vi "Get XNET Signal Names.vi"(6 "Add Info?":bool, 7 "Parent Ref in":T1 format="%.0x", 8 "error in":errorcluster, 9 "Tree In":refnum<vi>, 10 "Parent":string, 11 "Frms":refnum<k21>[](array[refnum])) -> (0 "error out":errorcluster, 1 "Tree Out":refnum<vi>, 3 "XNET Signal Names":refnum<k21>[](array[refnum]))   [LabVIEW 2015, in "Protection and Counter Addon System Explorer.lvlib"]
uses:
  Protection and Counter Addon System Explorer.lvlib
  <vilib>/NI Veristand/Custom Device API/Custom Device Item Ref.ctl
  <vilib>/NI Veristand/Custom Device API/Custom Device Channel.ctl
  <vilib>/NI Veristand/Custom Device API/Custom Device Channel Type.ctl
  Shared/SubVIs/GUID Lookup.vi
  <vilib>/NI Veristand/Custom Device API/Set Item Property (U32).vi
  <resource>/objmgr/xnet.rc
  <vilib>/NI VeriStand/Custom Device API/Custom Device API.lvlib
  Shared/Protection and Counter Addon Shared.lvlib
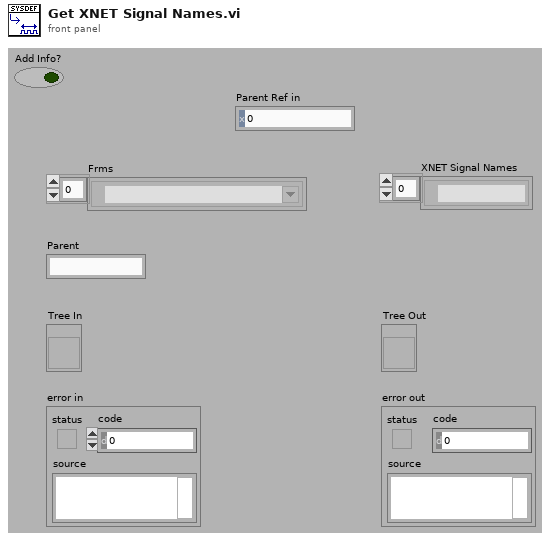
[diagram p1: front panel]
types:
  T1 = typedef "Custom Device API.lvlib/Custom Device Item Ref.ctl" = u64
  T2 = typedef "Custom Device API.lvlib/Custom Device Channel.ctl" = cluster{"Type":T3, "Units":string, "Default Value":dbl, "Faultable":bool, "Scalable":bool}
  T3 = typedef "Custom Device API.lvlib/Custom Device Channel Type.ctl" = enum16{"Input", "Output"}
  T4 = typedef "Custom Device API.lvlib/Custom Device Item Info.ctl" = cluster{"Name":string, "Is Channel":bool, "GUID":string, "Is Waveform":bool}
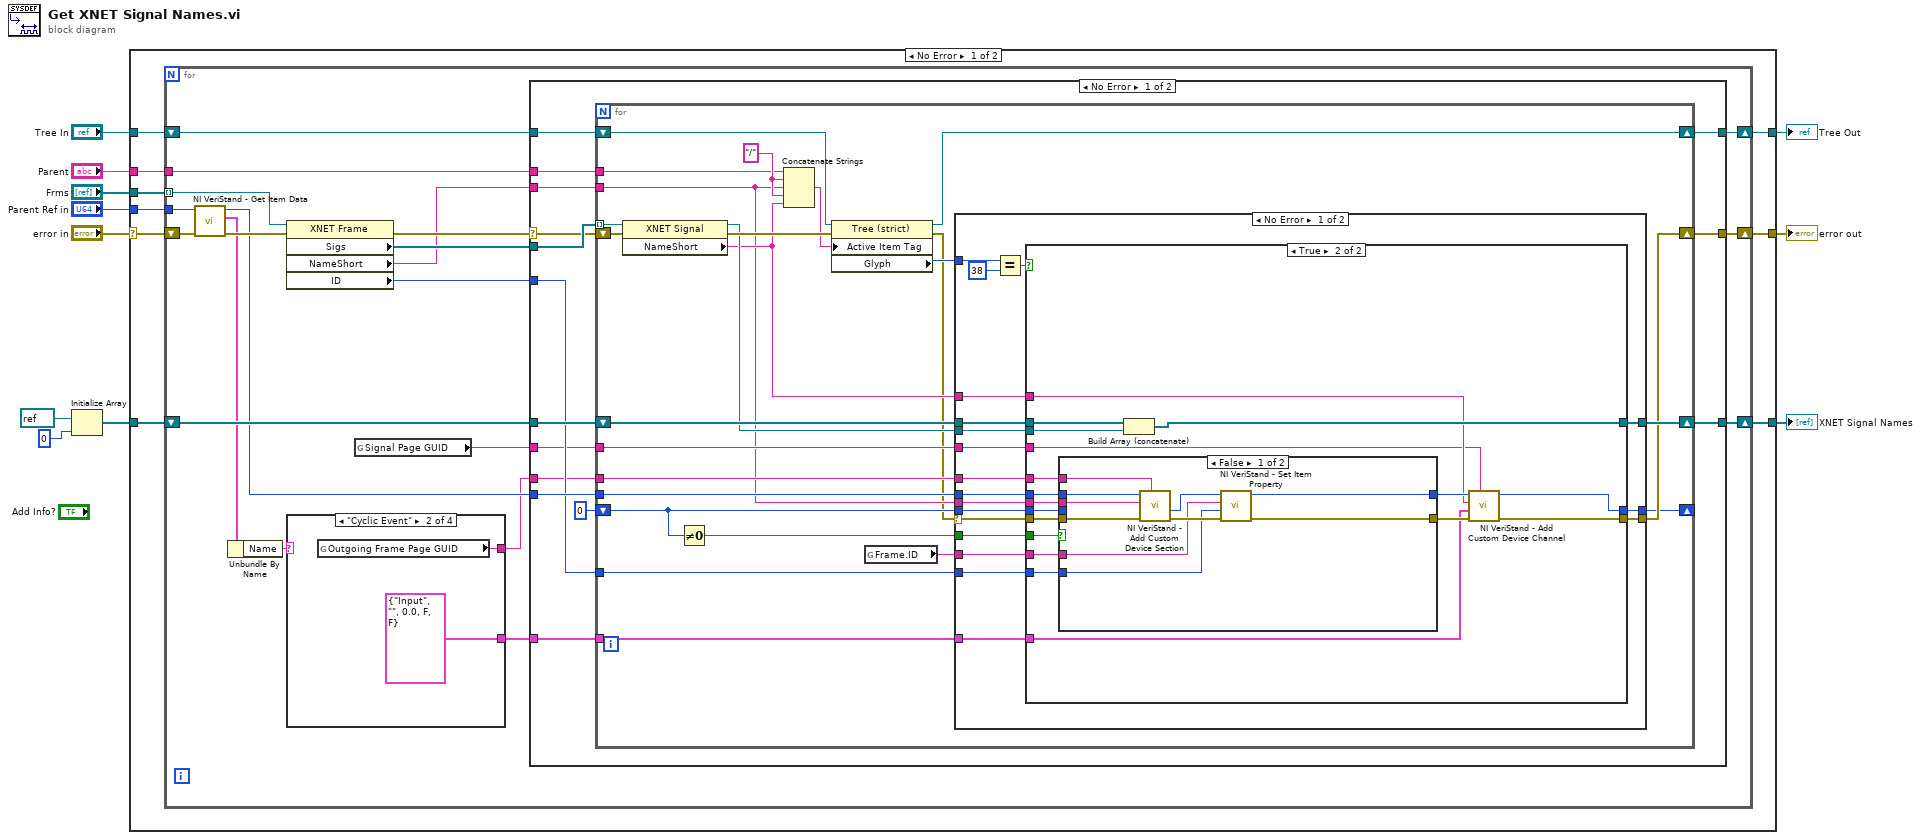
[diagram p0: block diagram]
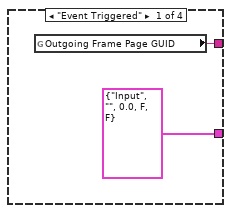
[diagram p2: hidden frame]
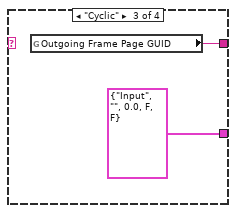
[diagram p3: hidden frame]
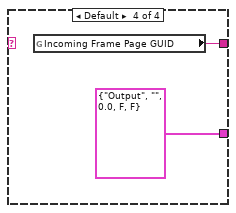
[diagram p4: hidden frame]
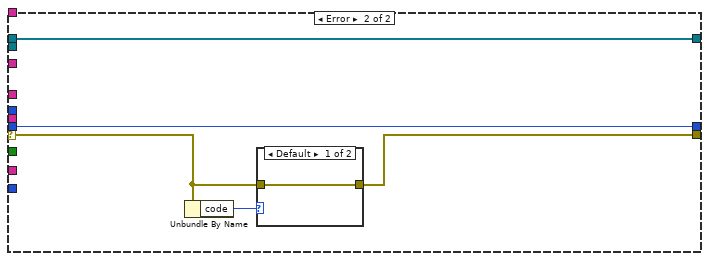
[diagram p7: hidden frame]
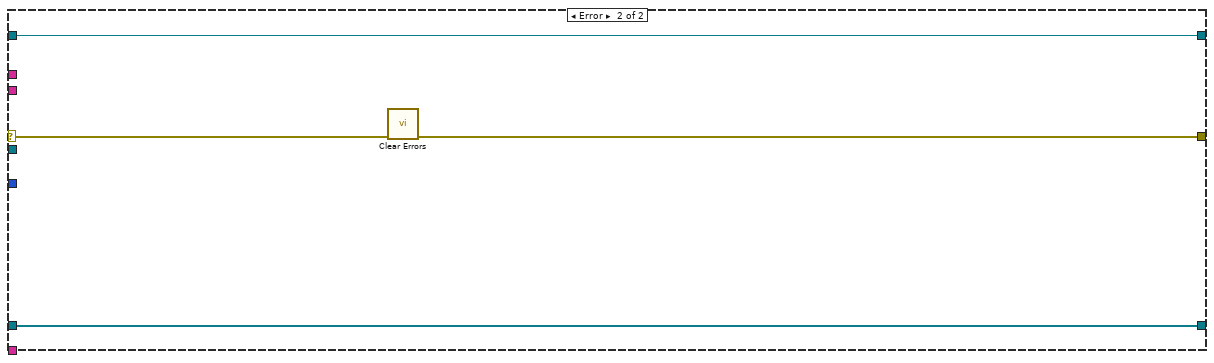
[diagram p9: hidden frame]
diagram:
  n1 = Initialize Array(refnum<k21> refnum ("XNET Signal"), 0 ("dimension size")) -> (w5:refnum<k21>[])
  n2 = case shown="No Error" "error in" {
    selector: "error in" -> [w17 w152]
    tunnel: "Parent" -> [w20 _]
    tunnel: [w19 w152] -> w10
    tunnel: "Frms" -> [w18 _]
    tunnel: [w16 _] -> w7
    tunnel: w5 -> [w15 _]
    tunnel: "Tree In" -> [w14 w151]
    tunnel: [w13 w151] -> w2
    tunnel: "Parent Ref in" -> [w12 _]
    frame No Error {
      n3 = for {
        shift-right: [w37] -> w19
        shift-left: w17 -> [w31]
        tunnel: w18 -> [w40] mode=indexing
        tunnel: w20 -> [w38]
        shift-right: [w34] -> w16
        shift-left: w15 -> [w35]
        shift-right: [w33] -> w13
        shift-left: w14 -> [w36]
        tunnel: w12 -> [w29]
        n4 = call <vilib>:"NI VeriStand - Get Item Data.vi"("error in (no error)"=w31, "Item Ref in"=w29) -> ("error out"=w30:errorcluster, "Item Info"=w27:T4, "Item Ref out"=w28:T1)  [unwired: 7 out]
        n5 = Unbundle By Name(w27) -> ("Name"=w26:string)
        n6 = property class="XNET Frame"(reference=w40, error in=w30) -> (error out=w32:errorcluster, "Sigs"=w39:refnum<k21>[], "NameShort"=w24:string, "ID"=w23:u32)  [unwired: 1 out]
        n7 = case shown="\"Cyclic Event\"" w26 {
          tunnel: [T2 {"Type"=enum."Input", "Units"="", "Default Value"=0.0, "Faultable"=FALSE, "Scalable"=FALSE} ("Channel") T2 {"Type"=enum."Input", "Units"="", "Default Value"=0.0, "Faultable"=FALSE, "Scalable"=FALSE} ("Channel") T2 {"Type"=enum."Input", "Units"="", "Default Value"=0.0, "Faultable"=FALSE, "Scalable"=FALSE} ("Channel") T2 {"Type"=enum."Output", "Units"="", "Default Value"=0.0, "Faultable"=FALSE, "Scalable"=FALSE} ("Channel")] -> w25
          tunnel: [w41 w43 w45 w47] -> w22
          frame "Event Triggered" {
            n8 = global read "GUID Lookup.vi" "Outgoing Frame Page GUID"() -> (w41:string)
          }
          frame "Cyclic Event" {
            n9 = global read "GUID Lookup.vi" "Outgoing Frame Page GUID"() -> (w43:string)
          }
          frame "Cyclic" {
            n10 = global read "GUID Lookup.vi" "Outgoing Frame Page GUID"() -> (w45:string)
          }
          frame Default {
            n11 = global read "GUID Lookup.vi" "Incoming Frame Page GUID"() -> (w47:string)
          }
        }
        n12 = global read "GUID Lookup.vi" "Signal Page GUID"() -> (w21:string)
        n13 = case shown="No Error" w32 {
          selector: w32 -> [w53 w147]
          tunnel: w39 -> [w63 _]
          tunnel: w24 -> [w62 _]
          tunnel: w38 -> [w61 _]
          tunnel: [w60 w148] -> w37
          tunnel: w36 -> [w59 w149]
          tunnel: w35 -> [w58 w150]
          tunnel: [w57 w150] -> w34
          tunnel: [w56 w149] -> w33
          tunnel: w28 -> [w55 _]
          tunnel: w23 -> [w52 _]
          tunnel: w21 -> [w51 _]
          tunnel: w22 -> [w50 _]
          tunnel: w25 -> [w49 _]
          frame No Error {
            n14 = for {
              tunnel: w63 -> [w88] mode=indexing
              tunnel: w62 -> [w66]
              tunnel: w61 -> [w85]
              shift-right: [w76] -> w60
              shift-left: w53 -> [w87]
              shift-right: [w80] -> w57
              shift-left: w58 -> [w79]
              shift-right: [w77] -> w56
              shift-left: w59 -> [w83]
              tunnel: w55 -> [w75]
              shift-right: [w74] -> _
              shift-left: T1 0 ("Parent Ref out") -> [w73]
              tunnel: w52 -> [w70]
              tunnel: w51 -> [w69]
              tunnel: w50 -> [w68]
              tunnel: w49 -> [w67]
              w86 = "/" ("string")
              n15 = property class="XNET Signal"(reference=w88, error in=w87) -> (reference out=w78:refnum<k21>, error out=w84:errorcluster, "NameShort"=w71:string)
              n16 = Not Equal To 0?(x=w73) -> (x != 0?=w72:bool)
              n17 = Concatenate Strings(w85, w86, w66, w86, w71) -> (w82:string)
              n18 = property class="Tree (strict)"(reference=w83, error in=w84, "Active Item Tag"=w82) -> (reference out=w77:refnum<vi>, error out=w65:errorcluster, "Glyph"=w81:i32)
              n19 = global read "GUID Lookup.vi" "Frame.ID"() -> (w64:string)
              n20 = case shown="No Error" w65 {
                selector: w65 -> [w89 w142]
                tunnel: w81 -> [w107 _]
                tunnel: [w104 w144] -> w80
                tunnel: w79 -> [w103 w144]
                tunnel: w78 -> [w102 _]
                tunnel: [w101 w141] -> w76
                tunnel: w75 -> [w100 _]
                tunnel: [w99 w145] -> w74
                tunnel: w73 -> [w98 w145]
                tunnel: w72 -> [w97 _]
                tunnel: w71 -> [w96 _]
                tunnel: w70 -> [w95 _]
                tunnel: w64 -> [w94 _]
                tunnel: w69 -> [w93 _]
                tunnel: w68 -> [w92 _]
                tunnel: w67 -> [w91 _]
                tunnel: w66 -> [w90 _]
                frame No Error {
                  n21 = Equal?(x=w107, y=38) -> (x = y?=w105:bool)
                  n22 = case shown="True" w105 {
                    tunnel: [w110 w126] -> w104
                    tunnel: w103 -> [w110 w128]
                    tunnel: w102 -> [_ w127]
                    tunnel: w97 -> [_ w125]
                    tunnel: w90 -> [_ w124]
                    tunnel: w89 -> [w109 w123]
                    tunnel: [w109 w111] -> w101
                    tunnel: w100 -> [_ w122]
                    tunnel: [w108 w119] -> w99
                    tunnel: w98 -> [w108 w121]
                    tunnel: w96 -> [_ w117]
                    tunnel: w92 -> [_ w116]
                    tunnel: w93 -> [_ w115]
                    tunnel: w95 -> [_ w114]
                    tunnel: w94 -> [_ w113]
                    tunnel: w91 -> [_ w112]
                    frame False {
                    }
                    frame True {
                      n23 = case shown="False" w125 {
                        tunnel: w124 -> [w138 _]
                        tunnel: w123 -> [w137 w140]
                        tunnel: [w130 w140] -> w120
                        tunnel: w122 -> [w136 _]
                        tunnel: [w129 w139] -> w118
                        tunnel: w121 -> [_ w139]
                        tunnel: w116 -> [w135 _]
                        tunnel: w114 -> [w131 _]
                        tunnel: w113 -> [w132 _]
                        frame False {
                          n24 = call <vilib>:"NI VeriStand - Add Custom Device Section.vi"("GUID (Default Section)"=w135, "error in (no error)"=w137, "Section Name"=w138, "Parent Ref in"=w136) -> ("error out"=w133:errorcluster, "Section Ptr"=w134:T1)  [unwired: 4 in, 2 out]
                          n25 = call-poly <vilib>:"NI VeriStand - Set Item Property.vi"("error in (no error)"=w133, "Value"=w131, "Property Name"=w132, "Item Ref in"=w134) -> ("error out"=w130:errorcluster, "Item Ref out"=w129:T1)  [unwired: 5 in, 1 out]
                        }
                        frame True {
                        }
                      }
                      n26 = Build Array (concatenate)(w128, w127) -> (w126:refnum<k21>[])
                      n27 = call <vilib>:"NI VeriStand - Add Custom Device Channel.vi"("GUID (Default Channel)"=w115, "error in (no error)"=w120, "Channel"=w112, "Channel Name"=w117, "Parent Ref in"=w118) -> ("error out"=w111:errorcluster, "Parent Ref out"=w119:T1)  [unwired: 3 in, 2 out]
                    }
                  }
                }
                frame Error {
                  n28 = Unbundle By Name(w142) -> ("code"=w143:i32)
                  n29 = case shown="Default" w143 {
                    tunnel: [w146 _] -> w141
                    tunnel: w142 -> [w146 _]
                    frame Default {
                    }
                    frame 1136 {
                    }
                  }
                }
              }
            }
          }
          frame Error {
            n30 = call <vilib>:"Clear Errors.vi"("error in (no error)"=w147) -> ("error out"=w148:errorcluster)  [unwired: 5 in, 1 out]
          }
        }
      }
    }
    frame Error {
    }
  }
  "error out" <- w10
  "XNET Signal Names" <- w7
  "Tree Out" <- w2
